vi "激光界面.vi"() -> ()   [LabVIEW 2021]
panel:
  in  ".NET容器 2":refnum<k24>(container)
  out "IsMarking":bool
  out "标刻内容":T1
  out "MES返回信息":T2
  out "执行状态":string
  out "MES状态":string
  in  "T 6":T3
  in  "T 5":T3
  in  "T 4":T3
  in  "T 3":T3
  in  "T 2":T3
  in  "T 1":T3
  in  "选项卡控件":enum32{"模板管理", "端口设置"}(tab)
  in  "产品选择 2":enum16{""}(ring)
  in  "删除":bool
  in  "新建 2":bool
  in  "产品选择":T4(radio)
  in  "刻码选择":enum32{"Item 0", "Item 1"}(radio)
  in  "模板文件路径":path
  out "添加的路径":path
  in  "手动标刻":bool
  in  "MES接口":cluster{"MES_IP":string, "端口":dbl}
  in  "扫码端口选择":refnum<visa-resource-name>
  # "9600 8 N 1"
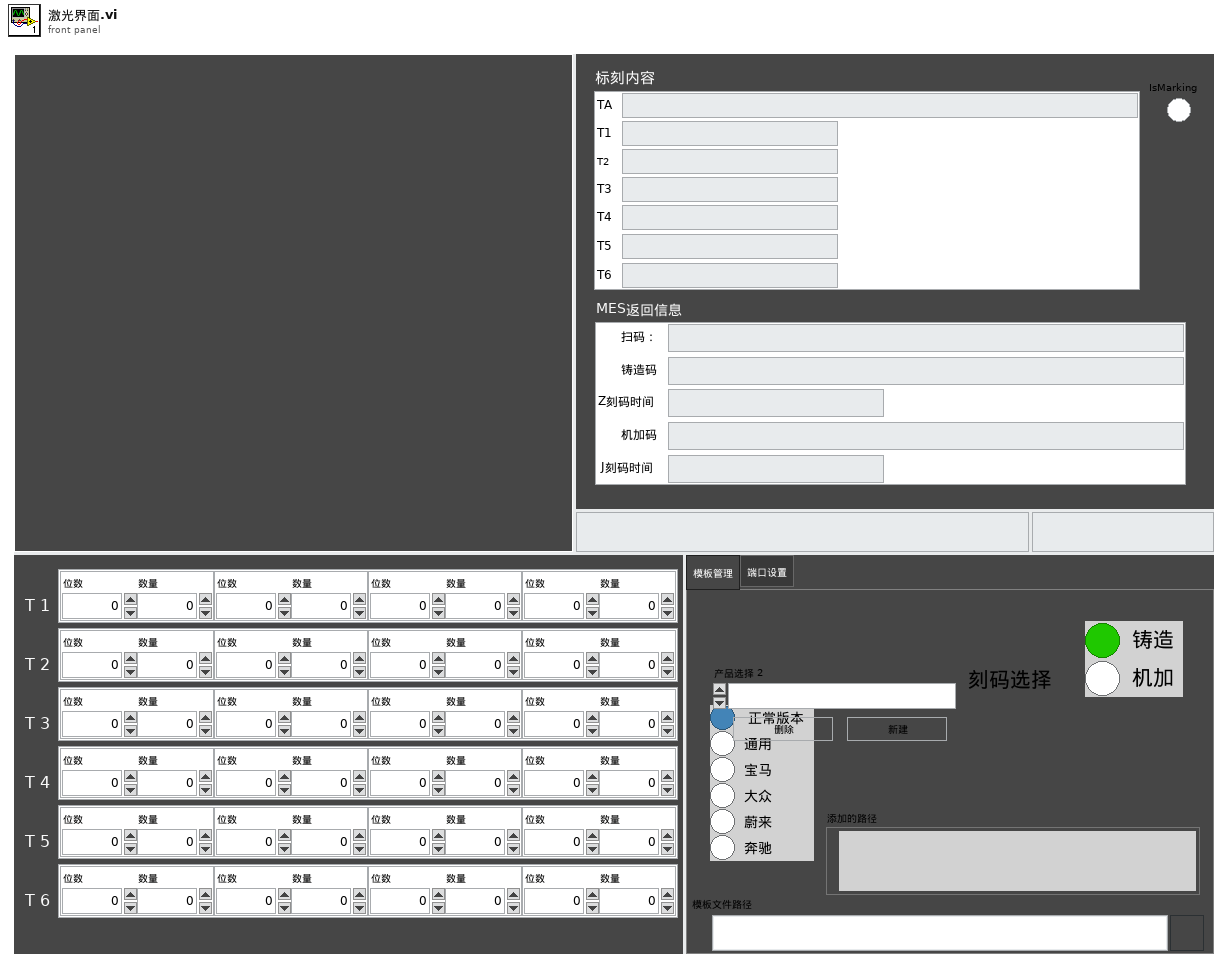
[diagram p1: front panel]
types:
  T1 = typedef "标刻内容.ctl" = cluster{"T1":string, "T2":string, "T3":string, "T4":string, "TA":string, "T5":string, "T6":string}
  T2 = typedef "MES返回二维码信息.ctl" = cluster{"扫码：":string, "铸造码":string, "Z刻码时间":string, "机加码":string, "J刻码时间":string}
  T3 = typedef "T码提取设置.ctl" = cluster{"T1 1":cluster{"位数":dbl, "数量":dbl}, "T1 2":cluster{"位数":dbl, "数量":dbl}, "T1 3":cluster{"位数":dbl, "数量":dbl}, "T1 4":cluster{"位数":dbl, "数量":dbl}}
  T4 = enum32{"Item 0", "Item 1", "宝马", "大众", "蔚来", "奔驰"}
  T5 = typedef "激光控制.ctl" = enum16{"初始化", "等待", "初始化激光", "加载模板", "替换字符", "启动刻码", "检测刻码完成", "停止标刻", "关闭调用", "释放", "退出"}
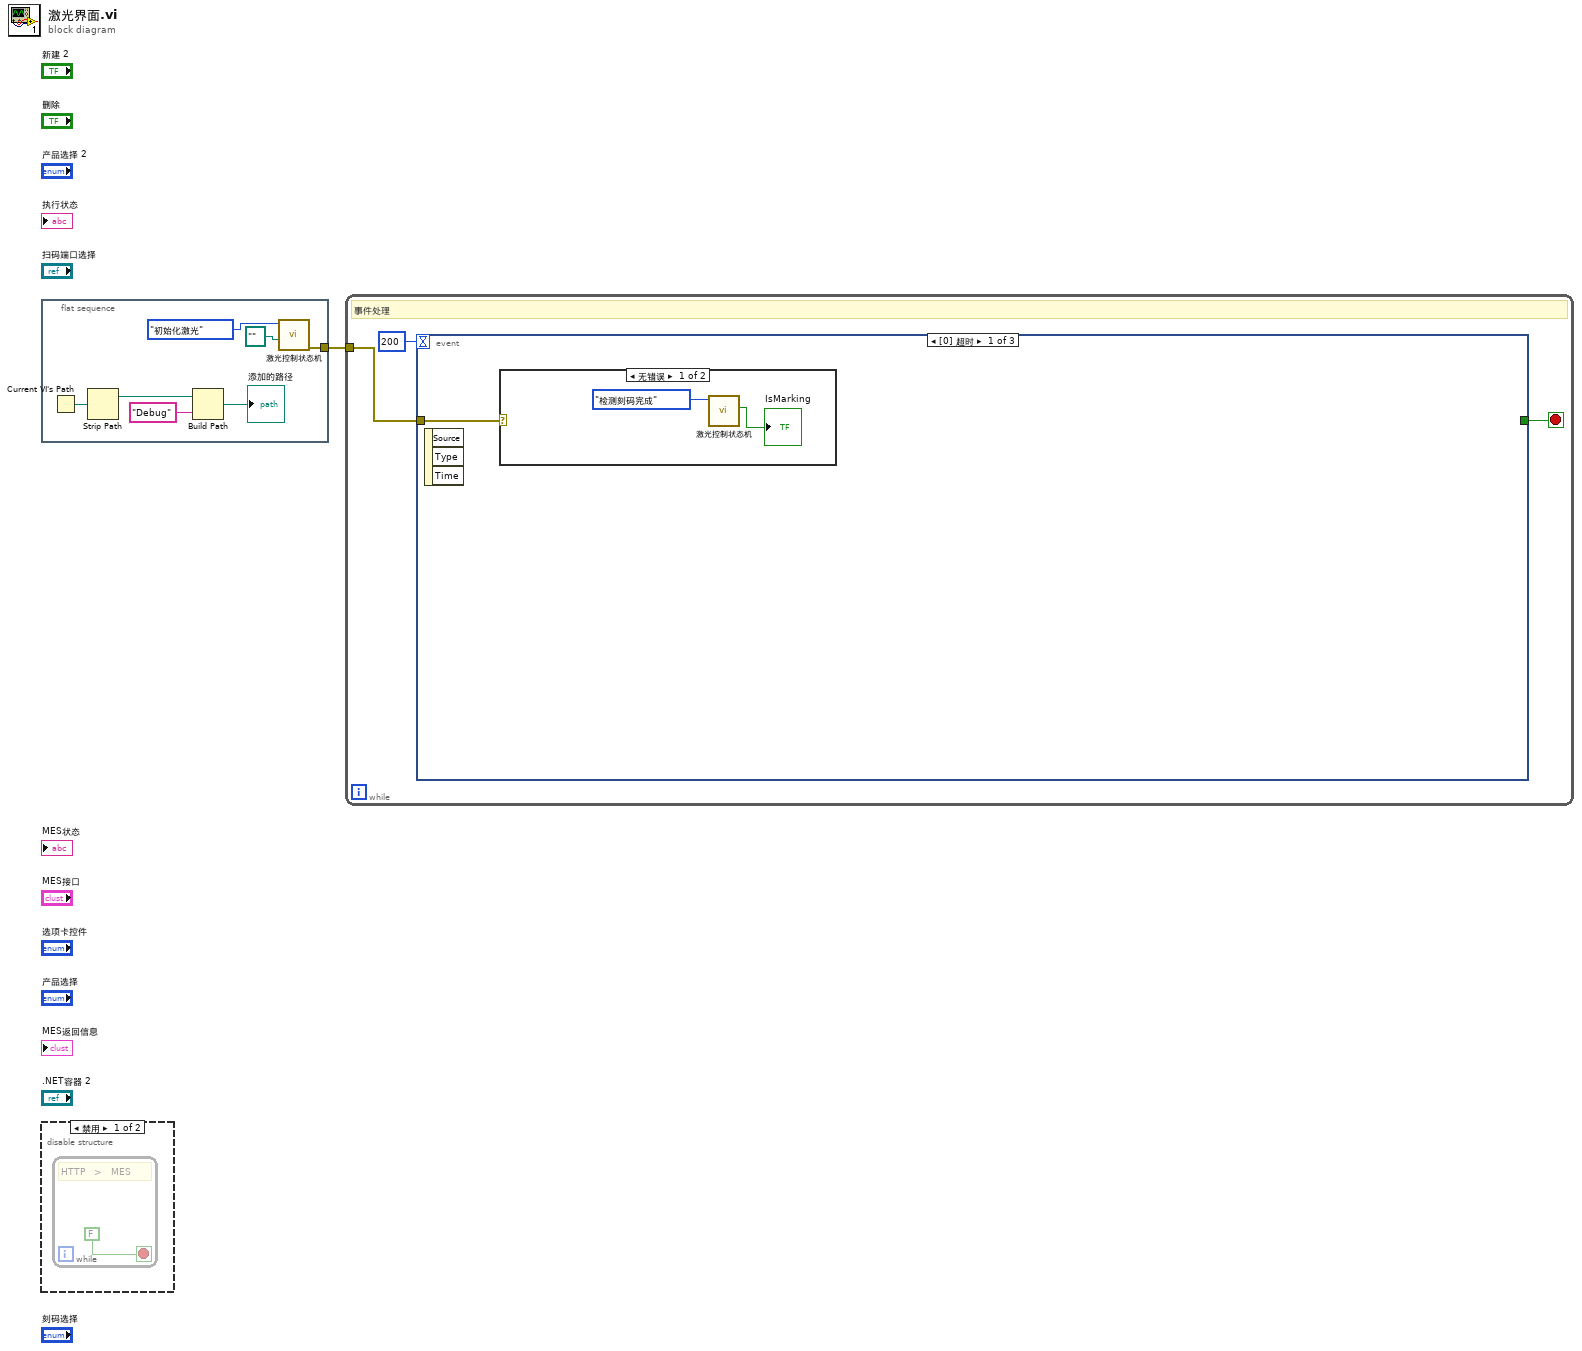
[diagram p0: block diagram]
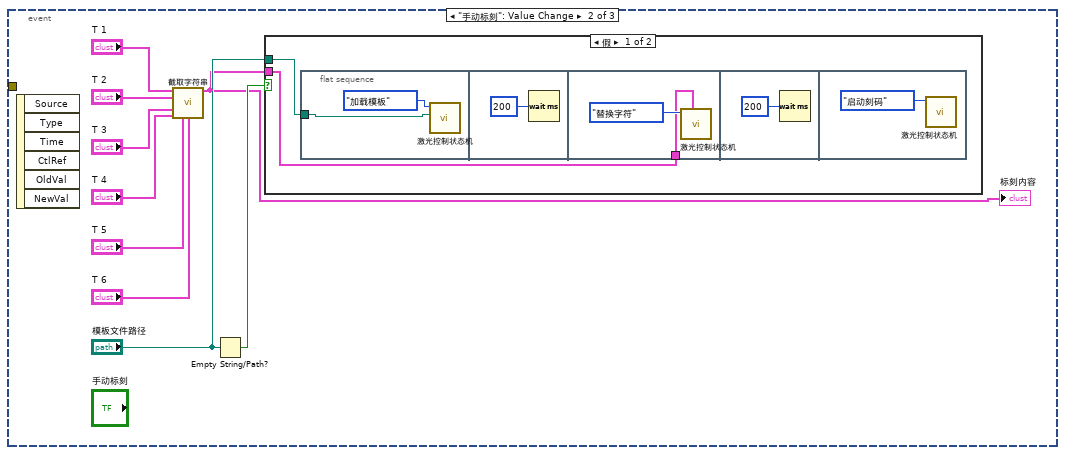
[diagram p4: hidden frame]
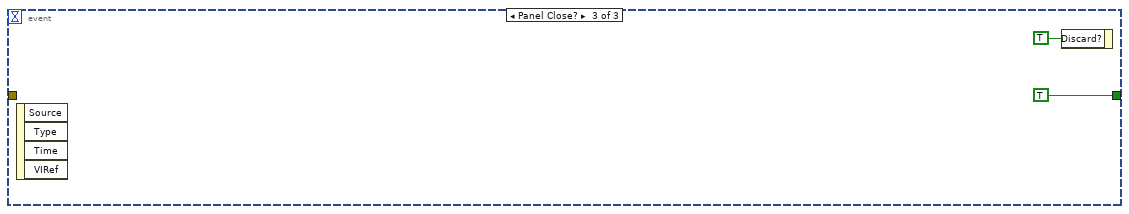
[diagram p6: hidden frame]
diagram:
  n1 = flat-sequence {
    tunnel: [w7] -> w1
    frame #0 {
      n2 = Current VI's Path() -> (path=w5:path)
      n3 = Strip Path(path=w5) -> (stripped path=w4:path)  [unwired: 1 out]
      n4 = Build Path(base path=w4, name or relative path="Debug") -> (appended path=→"添加的路径":path)
      n5 = call "激光控制状态机.vi"("debug项目路径"=path "", "激光控制"=激光控制."初始化激光") -> ("错误输出"=w7:errorcluster)  [unwired: 7 in, 2 out]
    }
  }
  n6 = disable-structure shown="禁用" {
    frame Disabled {
      n7 = while {
        stop <- FALSE stop-if-true
        # "HTTP   >   MES"
      }
    }
    frame Enabled {
    }
  }
  n8 = while {
    tunnel: w1 -> [w10]
    stop <- w12 stop-if-true
    # "事件处理"
    n9 = event shown="[0] 超时" {
      selector: _ -> [_ _ _]
      dyn-events: _ -> [_ _ _]
      timeout: 200 -> [_ _ _]
      tunnel: [_ _ TRUE] -> w12
      tunnel: w10 -> [w13 _ _]
      event Timeout {
        n10 = event-data() -> ()  [unwired: 1 in, 3 out]
        n11 = case shown="无错误" w13 {
          frame No Error {
            n12 = call "激光控制状态机.vi"("激光控制"=激光控制."检测刻码完成") -> ("IsMarking"=→"IsMarking":bool)  [unwired: 8 in, 2 out]
          }
          frame Error {
          }
        }
      }
      event "手动标刻": Value Change {
        n13 = event-data() -> ()  [unwired: 1 in, 6 out]
        n14 = call "截取字符串.vi"("T 1"="T 1", "T 2"="T 2", "T 3"="T 3", "T 4"="T 4", "T 5"="T 5", "T 6"="T 6") -> ("标刻内容"=w16:T1)  [unwired: 9 in]
        "标刻内容" <- w16
        n15 = Empty String/Path?(string/path="模板文件路径") -> (empty?=w23:bool)
        n16 = case shown="假" w23 {
          tunnel: "模板文件路径" -> [w26 _]
          tunnel: w16 -> [w25 _]
          frame False {
            n17 = flat-sequence {
              tunnel: w26 -> [w27]
              tunnel: w25 -> [w30]
              frame #0 {
                n18 = call "激光控制状态机.vi"("EZCAD模板路径"=w27, "激光控制"=激光控制."加载模板") -> ()  [unwired: 7 in, 3 out]
              }
              frame #1 {
                n19 = Wait (ms)(milliseconds to wait=u32 200 ("等待时间（毫秒）")) -> ()  [unwired: 1 out]
              }
              frame #2 {
                n20 = call "激光控制状态机.vi"("标刻内容"=w30, "激光控制"=激光控制."替换字符") -> ()  [unwired: 7 in, 3 out]
              }
              frame #3 {
                n21 = Wait (ms)(milliseconds to wait=u32 200 ("等待时间（毫秒）")) -> ()  [unwired: 1 out]
              }
              frame #4 {
                n22 = call "激光控制状态机.vi"("激光控制"=激光控制."启动刻码") -> ()  [unwired: 8 in, 3 out]
              }
            }
          }
          frame True {
          }
        }
      }
      event Panel Close? {
        n23 = event-data() -> ()  [unwired: 1 in, 4 out]
        n24 = event-data("Discard?"=TRUE ("放弃？")) -> ()  [unwired: 1 in, 1 out]
      }
    }
  }
